vi "XIS Setup Acquisition.vi"(8 "error in (no error)":errorcluster, 11 "ringBuffCount":i32) -> (0 "error out":errorcluster, 3 "function return":i32)   [LabVIEW 2022 SP3, in "VarexWrapper.lvlib"]
doc: "VAREX_API int XIS_SetupAcquisition();\n\nVAREX_API int XIS_SetupAcquisition(int ringBuffCount);"
uses:
  VarexWrapper.lvlib
  VarexWrapper.dll
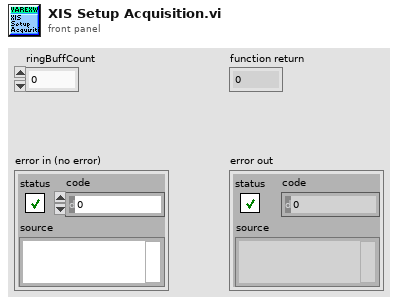
[diagram p1: front panel]
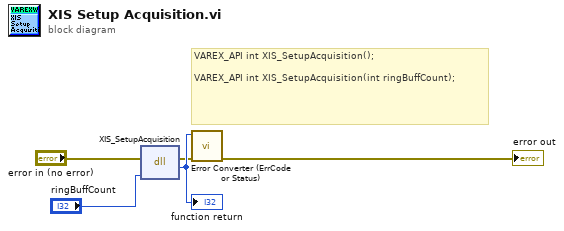
[diagram p0: block diagram]
diagram:
  # "VAREX_API int XIS_SetupAcquisition();\n\nVAREX_API int XIS_SetupAcquisition(int ringBuffCount);"
  n1 = dll-call lib="E:/SourceCodes/image-harvest/ImageHandler/VarexWrapperLvLib/VarexWrapper.*" fn="XIS_SetupAcquisition"(error in="error in (no error)", "ringBuffCount"="ringBuffCount") -> (error out=w2:errorcluster, w5:i32)  [unwired: 3 in, 1 out]
  "function return" <- w5
  n2 = call "Error Converter (ErrCode or Status).vi"("error in (no error)"=w2, "error code"=w5) -> ("error out"=→"error out":errorcluster)  [unwired: 9 in]
